vi "POC DAQmx.vi"() -> ()   [LabVIEW 2026]
uses:
  <vilib>/DAQmx/read.llb/DAQmx Read.vi
  <vilib>/DAQmx/read.llb/DAQmx Read (Analog 1D Wfm NChan NSamp).vi
  DAQ.lvlib
  My Singleton Module/My Singleton Module.lvlib
panel:
  out "data 2":waveform(dbl)[](graph) caption="data DQMH"
  in  "stop 2":bool
  out "data":waveform(dbl)[](graph)
  in  "stop":bool
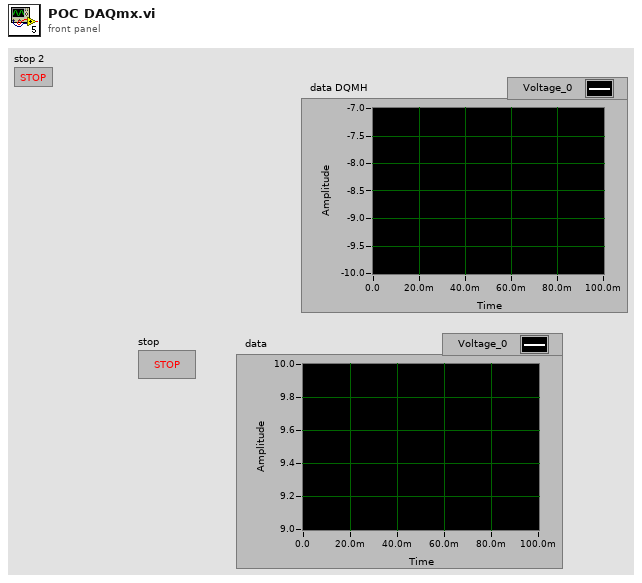
[diagram p1: front panel]
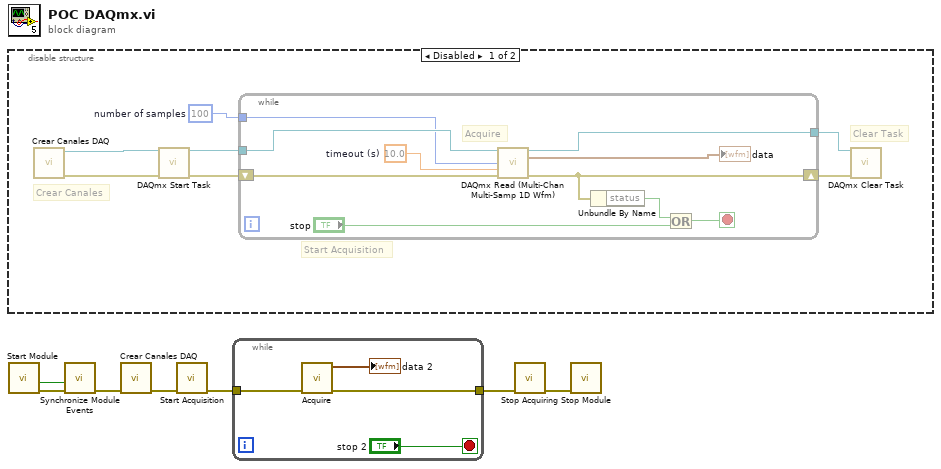
[diagram p0: block diagram]
diagram:
  n1 = disable-structure shown="Disabled" {
    frame Disabled {
      w12 = 100  # number of samples
      # "Clear Task"
      # "Start Acquisition"
      # "Crear Canales"
      n2 = call "Crear Canales DAQ.vi"() -> ("error out"=w8:errorcluster, "task out"=w9:refnum<k21>)  [unwired: 10 in]
      n3 = call <vilib>:"DAQmx Start Task.vi"("task/channels in"=w9, "error in"=w8) -> ("task out"=w14:refnum<k21>, "error out"=w13:errorcluster)  [unwired: 12 in]
      n4 = while {
        tunnel: w14 -> [w24]
        tunnel: w12 -> [w20]
        tunnel: [w21] -> w10
        shift-right: [w18] -> w11
        shift-left: w13 -> [w23]
        stop <- w17 stop-if-true
        w15 = 10.0  # timeout (s)
        # "Acquire"
        n5 = call-poly "DAQmx Read (Multi-Chan Multi-Samp 1D Wfm).vi"("task/channels in"=w24, "number of samples per channel"=w20, "timeout"=w15, "error in"=w23) -> ("task out"=w21:refnum<k21>, "data"=→"data":waveform(dbl)[], "error out"=w18:errorcluster)  [unwired: 9 in]
        n6 = Unbundle By Name(w18) -> ("status"=w19:bool)
        n7 = Or(x=w19, y="stop") -> (x .or. y?=w17:bool)
      }
      n8 = call <vilib>:"DAQmx Clear Task.vi"("task in"=w10, "error in"=w11) -> ()  [unwired: 13 in, 1 out]
    }
    frame Enabled {
    }
  }
  n9 = call "Start Module.vi"() -> ("error out"=w7:errorcluster, "Wait for Event Sync?"=w6:bool)  [unwired: 7 in, 3 out]
  n10 = call "Synchronize Module Events.vi"("error in"=w7, "Wait for Event Sync?"=w6) -> ("error out"=w5:errorcluster)  [unwired: 9 in]
  n11 = call "Crear Canales DAQ.vi"("error in"=w5) -> ("error out"=w4:errorcluster)  [unwired: 10 in]
  n12 = call "Start Acquisition.vi"("error in"=w4) -> ("error out"=w3:errorcluster)  [unwired: 10 in]
  n13 = while {
    tunnel: w3 -> [w28]
    tunnel: [w26] -> w2
    stop <- "stop 2" stop-if-true
    n14 = call "Acquire.vi"("error in"=w28) -> ("error out"=w26:errorcluster, "data"=→"data 2":waveform(dbl)[])  [unwired: 8 in, 1 out]
  }
  n15 = call "Stop Acquiring.vi"("error in"=w2) -> ("error out"=w1:errorcluster)  [unwired: 10 in]
  n16 = call "Stop Module.vi"("error in"=w1) -> ()  [unwired: 10 in, 1 out]
